vi "Host_main.vi"() -> ()   [LabVIEW 2025]
panel:
  out "Waveform Graph":i16[][](graph)
  in  "Stop":bool
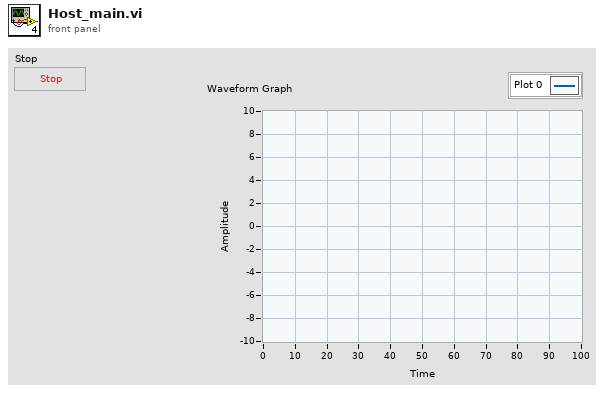
[diagram p1: front panel]
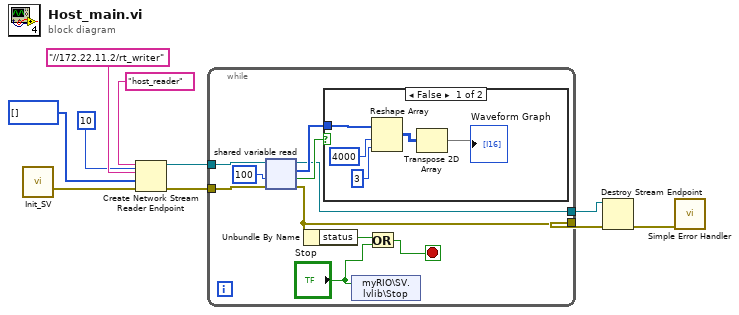
[diagram p0: block diagram]
diagram:
  n1 = call "Init_SV.vi"() -> ("error out"=w6:errorcluster)  [unwired: 11 in]
  n2 = Create Network Stream Reader Endpoint(7:10 ("reader buffer size"), 8:w6, 9:i16[] [], 10:"//172.22.11.2/rt_writer" ("writer url"), 11:"host_reader" ("writer name")) -> (0:w4:errorcluster, 3:w5:refnum<k21>)  [unwired: 2 in]
  n3 = while {
    tunnel: w5 -> [w20]
    tunnel: w4 -> [w19]
    tunnel: [w14] -> w3
    tunnel: [w11] -> w2
    stop <- w16 stop-if-true
    n4 = shared-variable-read(w20, w19, 100 ("timeout ms (-1)")) -> (w11:refnum<k21>, w14:errorcluster, w13:bool, w12:i16[])
    n5 = Unbundle By Name(w14) -> ("status"=w17:bool)
    n6 = case shown="False" w13 {
      tunnel: w12 -> [w25 _]
      frame False {
        n7 = Reshape Array(w25, 4000 ("dimension size"), 3 ("dimension size")) -> (w22:i16[][])
        n8 = Transpose 2D Array(2D array=w22) -> (transposed array=→"Waveform Graph":i16[][])
      }
      frame True {
      }
    }
    n9 = shared-variable "myRIO\\SV.lvlib\\Stop"("Stop") -> ()  [unwired: 1 in, 1 out]
    n10 = Or(x=w17, y="Stop") -> (x .or. y?=w16:bool)
  }
  n11 = Destroy Stream Endpoint(8:w3, 11:w2) -> (0:w1:errorcluster)
  n12 = call <vilib>:"Simple Error Handler.vi"("error in (no error)"=w1) -> ()  [unwired: 4 in, 5 out]
